vi "GOOP_DrawWirePreview_Simple.vi"(4 "Y-Offset":i16, 6 "X-Offset":i16, 9 "WireLength(100px)":i16=100, 10 "WireConfiguration":T1={"Edge thickness"=1, "Edge color"=6916708, "Center thickness"=1, "Center pattern"=enum."Solid", "CenterColor1"=8882055, "CenterColor2"=0, "Tunnels and terminals colors"=16711680}, 11 "PictureIn":picture) -> (1 "ImageHeight":i32, 2 "ImageWidth":i32, 3 "WirePictureOut":picture, 5 "ImageEnd-Y":i32, 7 "ImageEnd-X":i32)   [LabVIEW 2020]
uses:
  GOOP_WireConfigurationType.ctl
  GOOP_WirePattern.ctl
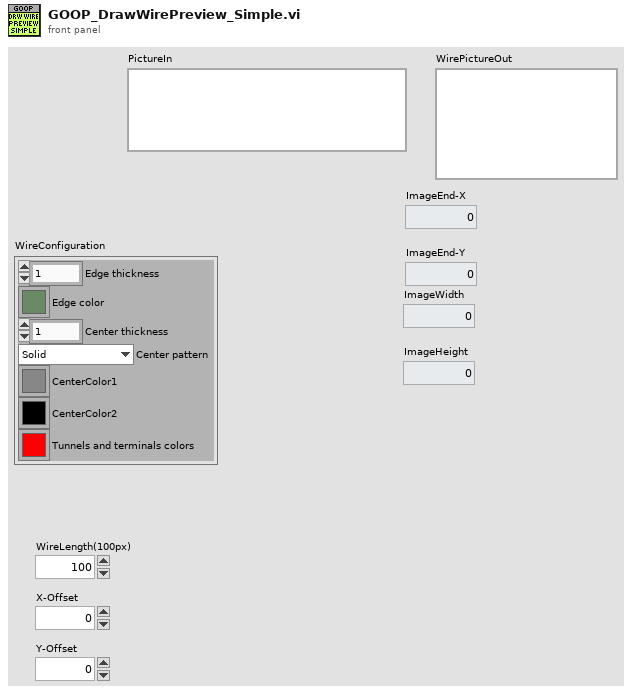
[diagram p1: front panel]
types:
  T1 = typedef "GOOP_WireConfigurationType.ctl" = cluster{"Edge thickness":i32, "Edge color":u32, "Center thickness":i32, "Center pattern":T2, "CenterColor1":u32, "CenterColor2":u32, "Tunnels and terminals colors":u32}
  T2 = typedef "GOOP_WirePattern.ctl" = enum16{"Solid", "Large dash", "Small dash"}
  T3 = cluster{"X-Offset":i16, "Y-Offset":i16, "X-Offset":i16, "Y-Offset":i16}
  T4 = typedef "imagedata.ctl" = cluster{"image type":i32, "image depth":i32, "image":u8[], "mask":u8[], "colors":u32[], "Rectangle":cluster{"left":i16, "top":i16, "right":i16, "bottom":i16}}
  T5 = cluster{"left":i16, "top":i16, "right":i16, "bottom":i16}
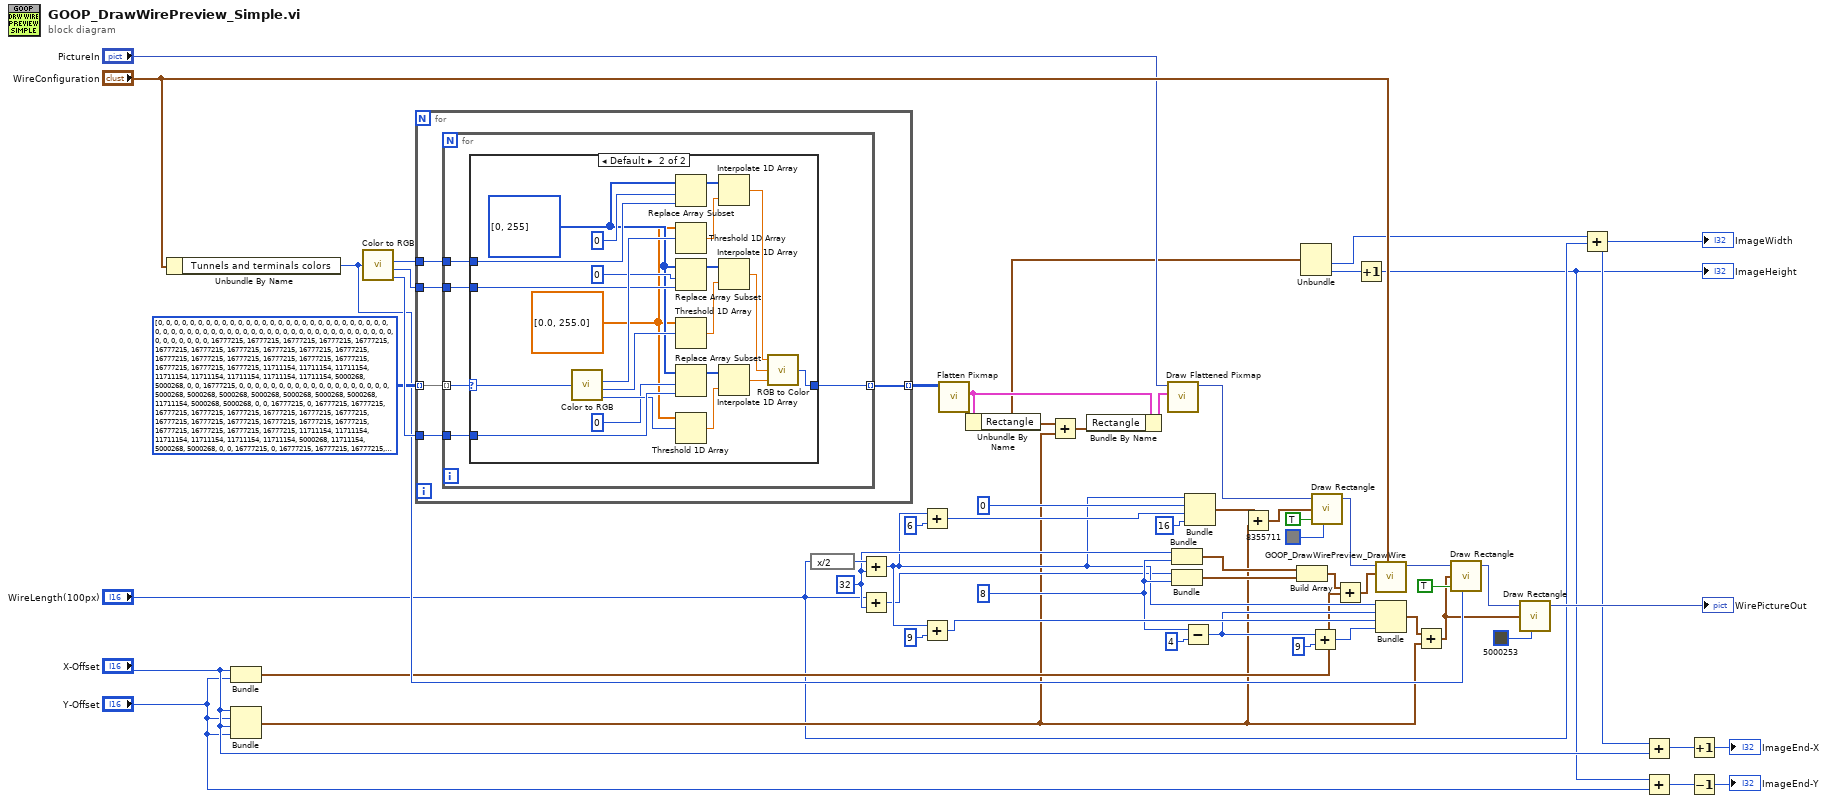
[diagram p0: block diagram]
diagram:
  w38 = i16 8 ("y")
  w27 = i16 32 ("x")
  n1 = Unbundle By Name("WireConfiguration") -> ("Tunnels and terminals colors"=w29:u32)
  n2 = Bundle("X-Offset"="X-Offset", "Y-Offset"="Y-Offset") -> (w24:cluster{"X-Offset":i16, "Y-Offset":i16})  [unwired: 1 in]
  n3 = Bundle("X-Offset"="X-Offset", "Y-Offset"="Y-Offset", "X-Offset"="X-Offset", "Y-Offset"="Y-Offset") -> (w15:T3)  [unwired: 1 in]
  n4 = call <vilib>:"Color to RGB.vi"("Color"=w29) -> ("R"=w57:u8, "G"=w56:u8, "B"=w55:u8)  [unwired: 1 out]
  n5 = for {
    tunnel: u32[][] [[0, 0, 0, 0, 0, 0, 0, 0, 0, 0, 0, 0, 0, 0, 0, 0, 0, 0, 0, 0, 0, 0, 0, 0, 0, 0, 0, 0, 0, 0, 0, 0], [0, 0, 0, 0, 0, 0, 0, 0, 0, 0, 0, 0, 0, 0, 0, 0, 0, 0, 0, 0, 0, 0, 0, 0, 0, 0, 0, 0, 0, 0, 0, 0], [0, 0, 16777215, 16777215, 16777215, 16777215, 16777215, 16777215, 16777215, 16777215, 16777215, 16777215, 16777215, 16777215, 16777215, 16777215, 16777215, 16777215, 16777215, 16777215, 16777215, 16777215, 11711154, 11711154, 11711154, 11711154, 11711154, 11711154, 11711154, 11711154, 5000268, 5000268], [0, 0, 16777215, 0, 0, 0, 0, 0, 0, 0, 0, 0, 0, 0, 0, 0, 0, 0, 0, 0, 0, 0, 5000268, 5000268, 5000268, 5000268, 5000268, 5000268, 5000268, 11711154, 5000268, 5000268], [0, 0, 16777215, 0, 16777215, 16777215, 16777215, 16777215, 16777215, 16777215, 16777215, 16777215, 16777215, 16777215, 16777215, 16777215, 16777215, 16777215, 16777215, 16777215, 16777215, 16777215, 11711154, 11711154, 11711154, 11711154, 11711154, 11711154, 5000268, 11711154, 5000268, 5000268], [0, 0, 16777215, 0, 16777215, 16777215, 16777215, 16777215, 16777215, 0, 0, 0, 16777215, 16777215, 0, 0, 0, 0, 16777215, 16777215, 16777215, 16777215, 5000268, 5000268, 11711154, 11711154, 11711154, 0, 5000268, 11711154, 5000268, 5000268], [0, 0, 16777215, 0, 16777215, 16777215, 16777215, 16777215, 0, 0, 16777215, 0, 0, 16777215, 0, 0, 16777215, 0, 0, 16777215, 16777215, 16777215, 5000268, 5000268, 11711154, 11711154, 11711154, 0, 0, 11711154, 5000268, 5000268], [0, 0, 16777215, 0, 16777215, 16777215, 16777215, 16777215, 0, 0, 16777215, 0, 0, 16777215, 0, 0, 0, 0, 16777215, 16777215, 16777215, 16777215, 5000268, 5000268, 11711154, 11711154, 11711154, 0, 0, 0, 5000268, 5000268], [0, 0, 16777215, 0, 16777215, 16777215, 16777215, 16777215, 0, 0, 16777215, 0, 0, 16777215, 0, 0, 16777215, 0, 0, 16777215, 0, 16777215, 5000268, 5000268, 11711154, 11711154, 11711154, 0, 0, 0, 5000268, 5000268], [0, 0, 16777215, 0, 16777215, 16777215, 16777215, 16777215, 0, 0, 16777215, 0, 0, 16777215, 0, 0, 16777215, 0, 0, 16777215, 0, 16777215, 5000268, 5000268, 11711154, 11711154, 11711154, 0, 0, 11711154, 5000268, 5000268], [0, 0, 16777215, 0, 16777215, 16777215, 16777215, 16777215, 16777215, 0, 0, 0, 16777215, 16777215, 0, 0, 0, 0, 16777215, 16777215, 16777215, 0, 5000268, 11711154, 11711154, 11711154, 11711154, 0, 5000268, 11711154, 5000268, 5000268], [0, 0, 16777215, 0, 16777215, 16777215, 16777215, 16777215, 16777215, 16777215, 16777215, 16777215, 16777215, 16777215, 16777215, 16777215, 16777215, 16777215, 16777215, 16777215, 16777215, 16777215, 11711154, 11711154, 11711154, 11711154, 11711154, 11711154, 5000268, 11711154, 5000268, 5000268], [0, 0, 16777215, 0, 0, 0, 0, 0, 0, 0, 0, 0, 0, 0, 0, 0, 0, 0, 0, 0, 0, 0, 5000268, 5000268, 5000268, 5000268, 5000268, 5000268, 5000268, 11711154, 5000268, 5000268], [0, 0, 16777215, 16777215, 16777215, 16777215, 16777215, 16777215, 16777215, 16777215, 16777215, 16777215, 16777215, 16777215, 16777215, 16777215, 16777215, 16777215, 16777215, 16777215, 16777215, 16777215, 11711154, 11711154, 11711154, 11711154, 11711154, 11711154, 11711154, 11711154, 5000268, 5000268], [0, 0, 0, 0, 0, 0, 0, 0, 0, 0, 0, 0, 0, 0, 0, 0, 0, 0, 0, 0, 0, 0, 0, 0, 0, 0, 0, 0, 0, 0, 0, 0], [0, 0, 0, 0, 0, 0, 0, 0, 0, 0, 0, 0, 0, 0, 0, 0, 0, 0, 0, 0, 0, 0, 0, 0, 0, 0, 0, 0, 0, 0, 0, 0]] ("24-bit pixmap") -> [w62] mode=indexing
    tunnel: w57 -> [w61]
    tunnel: w56 -> [w60]
    tunnel: w55 -> [w59]
    tunnel: [w58] -> w54 mode=indexing
    n6 = for {
      tunnel: w62 -> [w67] mode=indexing
      tunnel: w61 -> [w66]
      tunnel: w60 -> [w63]
      tunnel: w59 -> [w65]
      tunnel: [w64] -> w58 mode=indexing
      n7 = case shown="Default" w67 {
        selector: w67 -> [w68 w90]
        tunnel: w66 -> [_ w89]
        tunnel: w65 -> [_ w88]
        tunnel: [w68 w87] -> w64
        tunnel: w63 -> [_ w83]
        frame 16777215 {
        }
        frame Default {
          w72 = u8[] [0, 255]
          w71 = sgl[] [0.0, 255.0]
          n8 = call <vilib>:"Color to RGB.vi"("Color"=w90) -> ("R"=w86:u8, "G"=w85:u8, "B"=w84:u8)  [unwired: 1 out]
          n9 = Replace Array Subset(array=w72, new element=w89, index=0) -> (w81:u8[])
          n10 = Threshold 1D Array(2:w86, 3:w71) -> (0:w75:sgl)  [unwired: 1 in]
          n11 = Replace Array Subset(array=w72, new element=w83, index=0) -> (w79:u8[])
          n12 = Threshold 1D Array(2:w85, 3:w71) -> (0:w70:sgl)  [unwired: 1 in]
          n13 = Replace Array Subset(array=w72, new element=w88, index=0) -> (w76:u8[])
          n14 = Threshold 1D Array(2:w84, 3:w71) -> (0:w69:sgl)  [unwired: 1 in]
          n15 = Interpolate 1D Array(1:w75, 2:w81) -> (0:w80:dbl)
          n16 = Interpolate 1D Array(1:w70, 2:w79) -> (0:w74:dbl)
          n17 = Interpolate 1D Array(1:w69, 2:w76) -> (0:w73:dbl)
          n18 = call <vilib>:"RGB to Color.vi"("B"=w73, "G"=w74, "R"=w80) -> ("Color"=w87:u32)
        }
      }
    }
  }
  n19 = expression code="x/2"("WireLength(100px)") -> (w28:i16)
  n20 = Add(x=w28, y=w27) -> (x+y=w26:i16)
  n21 = Add(x="WireLength(100px)", y=w27) -> (x+y=w25:i16)
  n22 = Add(x=w26, y=i16 6) -> (x+y=w48:i16)
  n23 = Add(x=w26, y=i16 9) -> (x+y=w42:i16)
  n24 = call <vilib>:"Flatten Pixmap.vi"("24-bit pixmap"=w54) -> ("image data"=w17:T4)  [unwired: 10 in]
  n25 = Unbundle By Name(w17) -> ("Rectangle"=w12:T5)
  n26 = Add(x=w12, y=w15) -> (x+y=w13:cluster{i16, i16, i16, i16})
  n27 = Bundle By Name(cluster=w17, "Rectangle"=w13) -> (w16:T4)
  n28 = call <vilib>:"Draw Flattened Pixmap.vi"("image data"=w16, "picture"="PictureIn") -> ("new picture"=w51:picture)  [unwired: 7 in]
  n29 = Bundle("x"=w27, "y"=w38) -> (w40:cluster{"x":i16, "y":i16})  [unwired: 1 in]
  n30 = Bundle(w25, "y"=w38) -> (w39:cluster{i16, "y":i16})  [unwired: 1 in]
  n31 = Subtract(x=w38, y=i16 4) -> (x-y=w36:i16)
  n32 = Bundle(w26, "index"=i16 0, w48, "index"=i16 16) -> (w21:cluster{i16, "index":i16, i16, "index":i16})  [unwired: 1 in]
  n33 = Add(x=w21, y=w15) -> (x+y=w20:cluster{i16, i16, i16, i16})
  n34 = Build Array(w40, w39) -> (w23:cluster{"x":i16, "y":i16}[])
  n35 = Unbundle(w12) -> ("right"=w10:i16, "bottom"=w11:i16)  [unwired: 2 out]
  n36 = Add(x=w36, y=i16 9) -> (x+y=w34:i16)
  n37 = call <vilib>:"Draw Rectangle.vi"("picture"=w51, "rect"=w20, "fill?(F)"=TRUE, "color(black)"=u32 8355711) -> ("new picture"=w50:picture)  [unwired: 5 in]
  n38 = Add(x=w23, y=w24) -> (x+y=w22:cluster{i16, i16}[])
  n39 = Increment(x=w11) -> (x+1=w5:i16)
  "ImageHeight" <- w5
  n40 = call "GOOP_DrawWirePreview_DrawWire.vi"("WireConfiguration"="WireConfiguration", "Array"=w22, "PictureIn"=w50) -> ("PictureOut"=w32:picture)  [unwired: 8 in]
  n41 = Bundle(w26, w36, w42, w34) -> (w19:cluster{i16, i16, i16, i16})  [unwired: 1 in]
  n42 = Add(x=w19, y=w15) -> (x+y=w18:cluster{i16, i16, i16, i16})
  n43 = call <vilib>:"Draw Rectangle.vi"("picture"=w32, "rect"=w18, "fill?(F)"=TRUE, "color(black)"=w29) -> ("new picture"=w31:picture)  [unwired: 5 in]
  n44 = call <vilib>:"Draw Rectangle.vi"("picture"=w31, "rect"=w18, "color(black)"=u32 5000253) -> ("new picture"=→"WirePictureOut":picture)  [unwired: 6 in]
  n45 = Add(x=w10, y="WireLength(100px)") -> (x+y=w8:i16)
  "ImageWidth" <- w8
  n46 = Add(x=w8, y="X-Offset") -> (x+y=w6:i16)
  n47 = Add(x=w5, y="Y-Offset") -> (x+y=w3:i16)
  n48 = Increment(x=w6) -> (x+1=→"ImageEnd-X":i16)
  n49 = Decrement(x=w3) -> (x-1=→"ImageEnd-Y":i16)
